vi "Abort Sequence.vi"(8 "error in":errorcluster, 10 "Reason":string, 11 "Sequence Executor in":refnum<class "Sequence Executor.lvclass">) -> (0 "error out":errorcluster, 3 "Sequence Executor out":refnum<class "Sequence Executor.lvclass">)   [LabVIEW 2026, in "Sequence Executor.lvclass"]
doc: "Aborts the running sequence with Reason: the current step becomes ABORTED, Running false, Phase Idle, Overall Verdict ABORTED, Status shows Reason. When nothing runs only the Status changes. In both cases the plant is driven to the safe setpoints 0, 0, 0. Used by Stop Sequence.vi and Emergency Stop.vi."
uses:
  Sequence Executor.lvclass
  Sequence Executor.lvclass/Sequence Executor.ctl
  C:/Program Files/National Instruments/LabVIEW 2026/vi.lib/ActorFramework/Actor/Actor.lvclass
  C:/Users/DynaAdmin/PycharmProjects/Universal-sequence-executor-AF/src/Executor/Sequence Executor.lvclass
  <vilib>/ActorFramework/Message Enqueuer/Message Enqueuer.lvclass
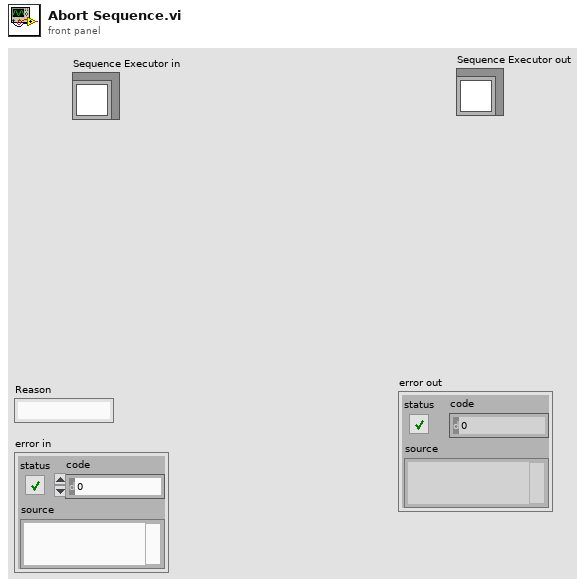
[diagram p1: front panel]
types:
  T1 = cluster{"pressure_sp_bar":dbl, "flow_sp_lpm":dbl, "displacement_sp_mm":dbl}
  T2 = typedef "Step Result.ctl" = cluster{"step_no":i32, "step_name":string, "result":string, "reason":string, "measured":dbl, "target":dbl, "duration_ms":dbl}
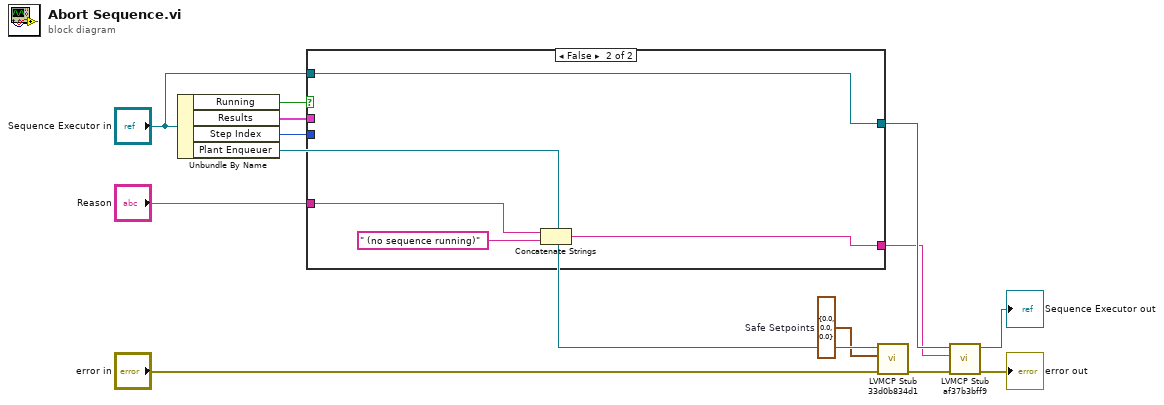
[diagram p0: block diagram]
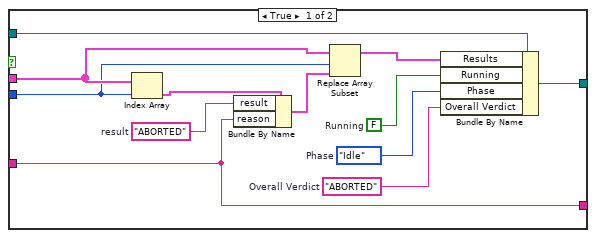
[diagram p2: hidden frame]
diagram:
  w7 = T1 {"pressure_sp_bar"=0.0, "flow_sp_lpm"=0.0, "displacement_sp_mm"=0.0}  # Safe Setpoints
  n1 = Unbundle By Name("Sequence Executor in") -> ("Running"=w9:bool, "Results"=w11:T2[], "Step Index"=w10:i32, "Plant Enqueuer"=w8:refnum<class "Message Enqueuer.lvclass">)
  n2 = case shown="False" w9 {
    tunnel: "Sequence Executor in" -> [w16 w27]
    tunnel: "Reason" -> [w14 w29]
    tunnel: w11 -> [w23 _]
    tunnel: w10 -> [w22 _]
    tunnel: [w15 w27] -> w5
    tunnel: [w14 w26] -> w4
    frame True {
      w17 = "ABORTED"  # Overall Verdict
      w18 = enum16{"Idle", "Settling", "Dwell", "Complete"}."Idle"  # Phase
      w19 = FALSE  # Running
      w25 = "ABORTED"  # result
      n3 = Index Array(array=w23, index=w22) -> (element=w24:T2)
      n4 = Bundle By Name(cluster=w24, "result"=w25, "reason"=w14) -> (w21:T2)
      n5 = Replace Array Subset(array=w23, new element=w21, index=w22) -> (w20:T2[])
      n6 = Bundle By Name(cluster=w16, "Results"=w20, "Running"=w19, "Phase"=w18, "Overall Verdict"=w17) -> (w15:refnum<class "Sequence Executor.lvclass">)
    }
    frame False {
      n7 = Concatenate Strings(w29, " (no sequence running)") -> (w26:string)
    }
  }
  n8 = call <userlib>:"LVMCP Stub 33d0b834d1.vi"("error in (no error)"="error in", "Plant Setpoints"=w7, "Message Enqueuer"=w8) -> ("error out"=w3:errorcluster)  [unwired: 7 in, 1 out]
  n9 = call <userlib>:"LVMCP Stub af37b3bff9.vi"("error in"=w3, "Status"=w4, "Sequence Executor in"=w5) -> ("error out"=→"error out":errorcluster, "Sequence Executor out"=→"Sequence Executor out":path)  [unwired: 7 in]
